vi "VariantToPlainText.vi"(7 "use system decimal point (T)":bool=TRUE, 11 "Variant-formatted Value":variant) -> (3 "String-formatted Value":string)   [LabVIEW 2013, in "OpenSerializer.lvlib" / "Serializer.PlainText.lvclass"]
uses:
  Serializer.PlainText.lvclass
  <vilib>/LabVIEW Open Source Project/Data Manipulation/TypeDescriptor/TypeDescriptor_GetName.vi
  <vilib>/LabVIEW Open Source Project/Data Manipulation/TypeDescriptor/TypeDescriptor_GetType.vi
  <vilib>/LabVIEW Open Source Project/Data Manipulation/TypeDescriptor/TypeDescriptor_GetPString.vi
  <vilib>/LabVIEW Open Source Project/Data Manipulation/Conversions/Flattened nD-Array to Flattened 1D-Array.vi
  <vilib>/Utility/VariantDataType/VariantType.lvlib
  <vilib>/LabVIEW Open Source Project/Data Manipulation/TypeDescriptor/OpenDescriptor.lvlib
  <vilib>/LabVIEW Open Source Project/Data Manipulation/Variant/OpenVariant.lvlib
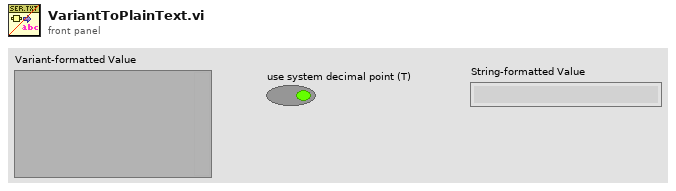
[diagram p1: front panel]
types:
  T1 = typedef "VariantType.lvlib/Type.ctl" = enum8{"Invalid Type", "Void", "I8", "I16", "I32", "I64", "U8", "U16", "U32", "U64", "Single Float", "Double Float", "Extended Float", "Single Complex", "Double Complex", "Extended Complex", "Enum U8", "Enum U16", "Enum U32", "Enum U64", "Single Float With Unit", "Double Float With Unit", "Extended Float With Unit", "Single Complex with Unit", "Double Complex with Unit", "Extended Complex with Unit", "Boolean", "String", "Path", "Picture", "Tag", "Array", "Cluster", "Variant", "LV Variant", "Waveform", "Timestamp", "Digital Waveform", "Digital Data", "ExpressData", "Refnum", "External Data", "VI", "Poly VI", "LabVIEW Class Instance", "Fixed Point"}
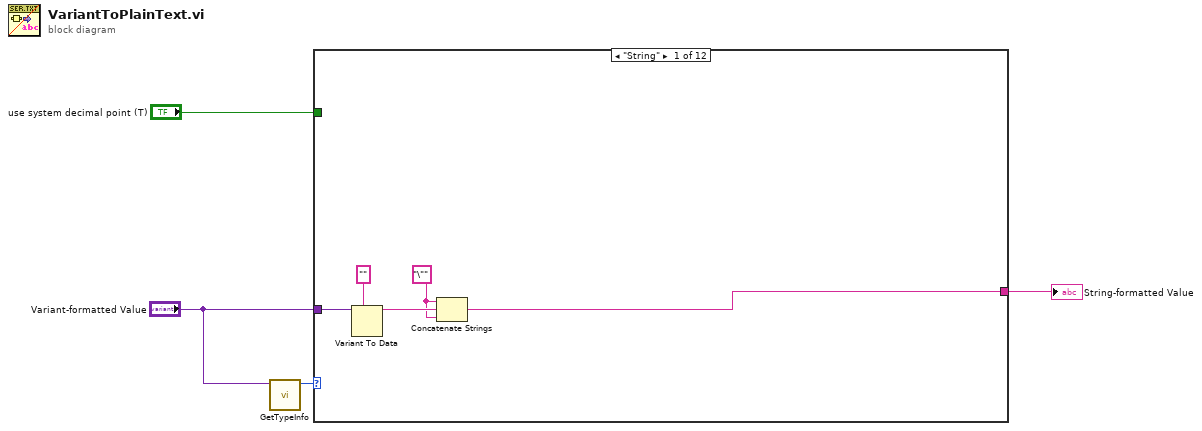
[diagram p0: block diagram]
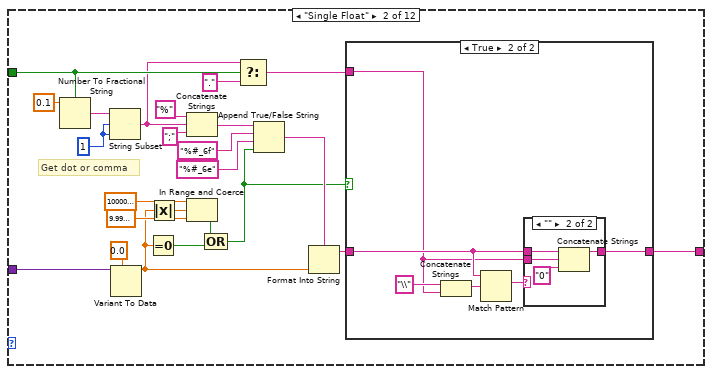
[diagram p2: hidden frame]
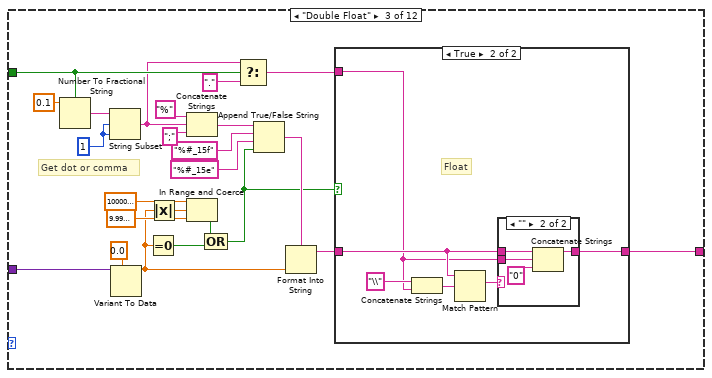
[diagram p5: hidden frame]
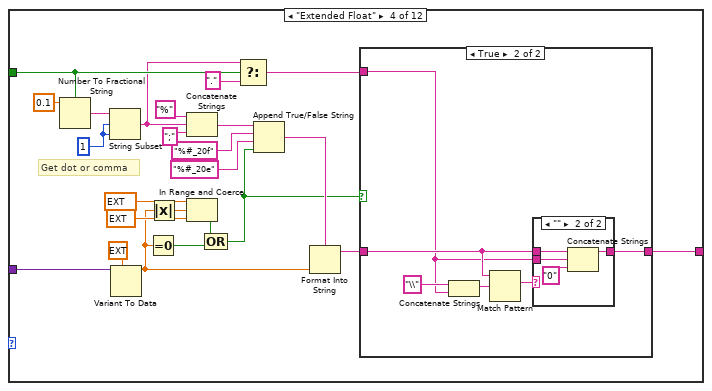
[diagram p8: hidden frame]
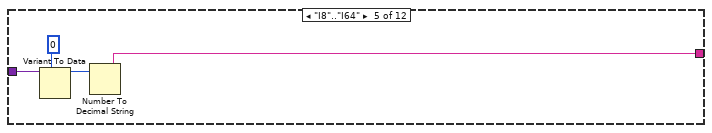
[diagram p11: hidden frame]
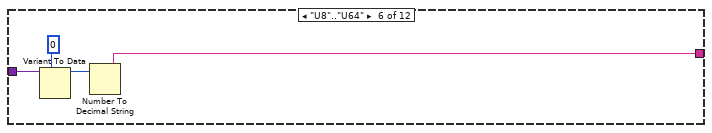
[diagram p12: hidden frame]
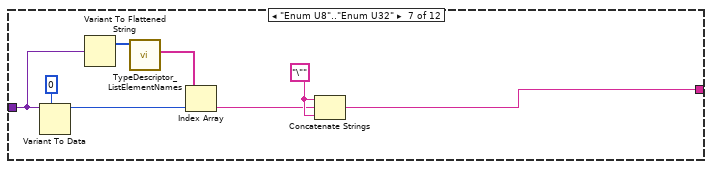
[diagram p13: hidden frame]
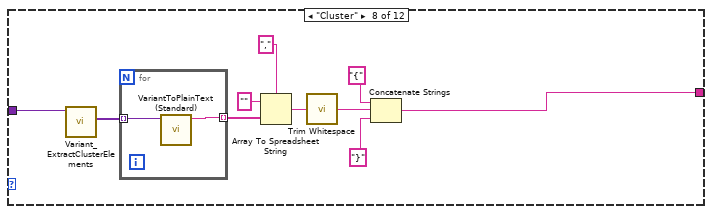
[diagram p14: hidden frame]
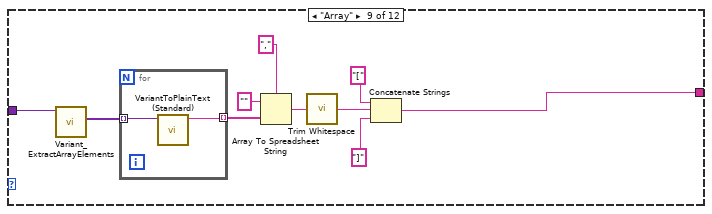
[diagram p15: hidden frame]
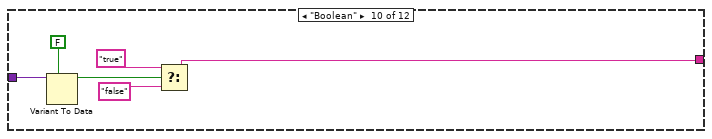
[diagram p16: hidden frame]
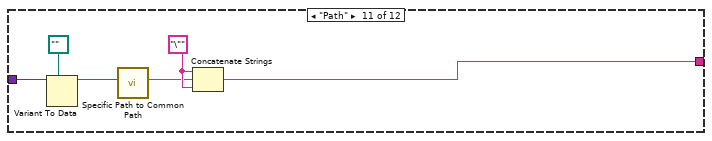
[diagram p17: hidden frame]
diagram:
  n1 = call <vilib>:"GetTypeInfo.vi"("Variant"="Variant-formatted Value") -> ("Type Enum"=w4:T1)  [unwired: 6 in, 4 out]
  n2 = case shown="\"String\"" w4 {
    tunnel: "Variant-formatted Value" -> [w9 w27 w63 w99 w119 w123 w132 w140 w147 w163 w169 _]
    tunnel: [w6 w16 w52 w88 w118 w122 w126 w142 w154 w160 w166 _] -> w1
    tunnel: "use system decimal point (T)" -> [_ w15 w51 w87 _ _ _ _ _ _ _ _]
    frame "String" {
      w5 = "\"" ("Format String")
      n3 = Variant To Data(type="" ("Format String"), Variant=w9) -> (data=w7:string)  [unwired: 1 in, 1 out]
      n4 = Concatenate Strings(w5, w7, w5) -> (w6:string)
    }
    frame "Single Float" {
      w24 = 1 ("length (rest)")
      # "Get dot or comma"
      n5 = Number To Fractional String(use system decimal point (T)=w15, number=0.1) -> (F-format string=w25:string)  [unwired: 2 in]
      n6 = String Subset(string=w25, offset (0)=w24, length (rest)=w24) -> (substring=w13:string)
      n7 = Variant To Data(type=sgl 0.0, Variant=w27) -> (data=w18:sgl)  [unwired: 1 in, 1 out]
      n8 = Equal To 0?(x=w18) -> (x = 0?=w29:bool)
      n9 = Absolute Value(x=w18) -> (abs(x)=w30:sgl)
      n10 = Concatenate Strings("%" ("format string"), w13, ";" ("format string")) -> (w21:string)
      n11 = In Range and Coerce(upper limit=sgl 1000000.0, x=w30, lower limit=sgl 0.0001 ("upper limit")) -> (In Range?=w28:bool)  [unwired: 1 out]
      n12 = Compound Arithmetic op=OR(w28, w29) -> (w10:bool)
      n13 = Select(t=w13, s=w15, f="." ("regular expression")) -> (s? t:f=w11:string)
      n14 = Append True/False String(1:w10, 2:"%#_6e" ("format string"), 3:"%#_6f" ("format string"), 4:w21) -> (0:w17:string)
      n15 = Format Into String(format string=w17, w18) -> (resulting string=w12:string)  [unwired: 2 in, 1 out]
      n16 = case shown="True" w10 {
        tunnel: [w34 w40] -> w16
        tunnel: w12 -> [w34 w38]
        tunnel: w11 -> [_ w36]
        frame False {
        }
        frame True {
          n17 = Concatenate Strings("\\" ("string"), w36) -> (w35:string)
          n18 = Match Pattern(string=w38, regular expression=w35) -> (match substring=w39:string)  [unwired: 1 in, 3 out]
          n19 = case shown="\"\"" w39 {
            tunnel: w38 -> [w41 w44]
            tunnel: [w41 w45] -> w40
            tunnel: w36 -> [_ w42]
            frame Default {
            }
            frame "" {
              n20 = Concatenate Strings(w44, w42, "0" ("regular expression")) -> (w45:string)
            }
          }
        }
      }
    }
    frame "Double Float" {
      w60 = 1 ("length (rest)")
      # "Get dot or comma"
      n21 = Number To Fractional String(use system decimal point (T)=w51, number=0.1) -> (F-format string=w61:string)  [unwired: 2 in]
      n22 = String Subset(string=w61, offset (0)=w60, length (rest)=w60) -> (substring=w49:string)
      n23 = Variant To Data(type=0.0, Variant=w63) -> (data=w54:dbl)  [unwired: 1 in, 1 out]
      n24 = Equal To 0?(x=w54) -> (x = 0?=w65:bool)
      n25 = Absolute Value(x=w54) -> (abs(x)=w66:dbl)
      n26 = Concatenate Strings("%" ("format string"), w49, ";" ("format string")) -> (w57:string)
      n27 = In Range and Coerce(upper limit=1000000.0, x=w66, lower limit=9.999999747378752e-05 ("upper limit")) -> (In Range?=w64:bool)  [unwired: 1 out]
      n28 = Compound Arithmetic op=OR(w64, w65) -> (w46:bool)
      n29 = Select(t=w49, s=w51, f="." ("regular expression")) -> (s? t:f=w47:string)
      n30 = Append True/False String(1:w46, 2:"%#_15e" ("format string"), 3:"%#_15f" ("format string"), 4:w57) -> (0:w53:string)
      n31 = Format Into String(format string=w53, w54) -> (resulting string=w48:string)  [unwired: 2 in, 1 out]
      n32 = case shown="True" w46 {
        tunnel: [w70 w76] -> w52
        tunnel: w48 -> [w70 w74]
        tunnel: w47 -> [_ w72]
        frame False {
          # "Exponential"
        }
        frame True {
          # "Float"
          n33 = Concatenate Strings("\\" ("string"), w72) -> (w71:string)
          n34 = Match Pattern(string=w74, regular expression=w71) -> (match substring=w75:string)  [unwired: 1 in, 3 out]
          n35 = case shown="\"\"" w75 {
            tunnel: w74 -> [w77 w80]
            tunnel: [w77 w81] -> w76
            tunnel: w72 -> [_ w78]
            frame Default {
            }
            frame "" {
              n36 = Concatenate Strings(w80, w78, "0" ("regular expression")) -> (w81:string)
            }
          }
        }
      }
    }
    frame "Extended Float" {
      w96 = 1 ("length (rest)")
      # "Get dot or comma"
      n37 = Number To Fractional String(use system decimal point (T)=w87, number=0.1) -> (F-format string=w97:string)  [unwired: 2 in]
      n38 = String Subset(string=w97, offset (0)=w96, length (rest)=w96) -> (substring=w84:string)
      n39 = Variant To Data(type=ext 0.0, Variant=w99) -> (data=w90:ext)  [unwired: 1 in, 1 out]
      n40 = Equal To 0?(x=w90) -> (x = 0?=w101:bool)
      n41 = Absolute Value(x=w90) -> (abs(x)=w102:ext)
      n42 = Concatenate Strings("%" ("format string"), w84, ";" ("format string")) -> (w93:string)
      n43 = In Range and Coerce(upper limit=ext 1000000.0, x=w102, lower limit=ext 9.999999747378752e-05 ("upper limit")) -> (In Range?=w100:bool)  [unwired: 1 out]
      n44 = Compound Arithmetic op=OR(w100, w101) -> (w82:bool)
      n45 = Select(t=w84, s=w87, f="." ("regular expression")) -> (s? t:f=w83:string)
      n46 = Append True/False String(1:w82, 2:"%#_20e" ("format string"), 3:"%#_20f" ("format string"), 4:w93) -> (0:w89:string)
      n47 = Format Into String(format string=w89, w90) -> (resulting string=w86:string)  [unwired: 2 in, 1 out]
      n48 = case shown="True" w82 {
        tunnel: [w106 w112] -> w88
        tunnel: w86 -> [w106 w110]
        tunnel: w83 -> [_ w108]
        frame False {
        }
        frame True {
          n49 = Concatenate Strings("\\" ("string"), w108) -> (w107:string)
          n50 = Match Pattern(string=w110, regular expression=w107) -> (match substring=w111:string)  [unwired: 1 in, 3 out]
          n51 = case shown="\"\"" w111 {
            tunnel: w110 -> [w113 w116]
            tunnel: [w113 w117] -> w112
            tunnel: w108 -> [_ w114]
            frame Default {
            }
            frame "" {
              n52 = Concatenate Strings(w116, w114, "0" ("regular expression")) -> (w117:string)
            }
          }
        }
      }
    }
    frame "I8".."I64" {
      n53 = Variant To Data(type=i64 0, Variant=w119) -> (data=w120:i64)  [unwired: 1 in, 1 out]
      n54 = Number To Decimal String(number=w120) -> (decimal integer string=w118:string)  [unwired: 1 in]
    }
    frame "U8".."U64" {
      n55 = Variant To Data(type=u64 0, Variant=w123) -> (data=w124:u64)  [unwired: 1 in, 1 out]
      n56 = Number To Decimal String(number=w124) -> (decimal integer string=w122:string)  [unwired: 1 in]
    }
    frame "Enum U8".."Enum U32" {
      w128 = "\"" ("Format String")
      n57 = Variant To Data(type=0, Variant=w132) -> (data=w129:i32)  [unwired: 1 in, 1 out]
      n58 = Variant To Flattened String(Variant=w132) -> (1:w131:i16[])  [unwired: 1 out]
      n59 = call <vilib>:"TypeDescriptor_ListElementNames.vi"("type descriptor"=w131) -> ("element names"=w130:string[])  [unwired: 7 in, 3 out]
      n60 = Index Array(array=w130, index=w129) -> (element=w127:string)
      n61 = Concatenate Strings(w128, w127, w128) -> (w126:string)
    }
    frame "Cluster" {
      n62 = call <vilib>:"Variant_ExtractClusterElements.vi"("Cluster"=w140) -> ("Elements"=w139:variant[])  [unwired: 8 in, 2 out]
      n63 = for {
        tunnel: w139 -> [w145] mode=indexing
        tunnel: [w144] -> w138 mode=indexing
        n64 = call "VariantToPlainText (Standard).vi"("Variant-formatted Value"=w145) -> ("String-formatted Value"=w144:string)  [unwired: 10 in]
      }
      n65 = Array To Spreadsheet String(delimiter (Tab)="," ("Format String"), array=w138, 3:"" ("format string")) -> (spreadsheet string=w135:string)
      n66 = call <vilib>:"Trim Whitespace.vi"("string"=w135) -> ("trimmed string"=w134:string)  [unwired: 1 in]
      n67 = Concatenate Strings("{" ("Format String"), w134, "}" ("Format String")) -> (w142:string)
    }
    frame "Array" {
      n68 = call <vilib>:"Variant_ExtractArrayElements.vi"("Array"=w147) -> ("Elements"=w146:variant[])  [unwired: 7 in, 3 out]
      n69 = for {
        tunnel: w146 -> [w157] mode=indexing
        tunnel: [w156] -> w152 mode=indexing
        n70 = call "VariantToPlainText (Standard).vi"("Variant-formatted Value"=w157) -> ("String-formatted Value"=w156:string)  [unwired: 10 in]
      }
      n71 = Array To Spreadsheet String(delimiter (Tab)="," ("Format String"), array=w152, 3:"" ("format string")) -> (spreadsheet string=w149:string)
      n72 = call <vilib>:"Trim Whitespace.vi"("string"=w149) -> ("trimmed string"=w148:string)  [unwired: 1 in]
      n73 = Concatenate Strings("[" ("Format String"), w148, "]" ("Format String")) -> (w154:string)
    }
    frame "Boolean" {
      n74 = Variant To Data(type=FALSE, Variant=w163) -> (data=w161:bool)  [unwired: 1 in, 1 out]
      n75 = Select(t="true", s=w161, f="false") -> (s? t:f=w160:string)
    }
    frame "Path" {
      w167 = "\"" ("Format String")
      n76 = Variant To Data(type=path "" ("Format String"), Variant=w169) -> (data=w165:path)  [unwired: 1 in, 1 out]
      n77 = call "Specific Path to Common Path.vi"("specific path"=w165) -> ("common path"=w164:string)  [unwired: 10 in]
      n78 = Concatenate Strings(w167, w164, w167) -> (w166:string)
    }
    frame Default {
    }
  }
  "String-formatted Value" <- w1
